vi "Initialize.vi"(8 "error in (no error)":errorcluster, 10 "logger name":string, 11 "file handler in":refnum<class "File Handler.lvclass">) -> (0 "error out":errorcluster, 2 "handler name":string, 3 "file handler out":refnum<class "File Handler.lvclass">)   [LabVIEW 2018, in "GLog.lvlib" / "File Handler.lvclass"]
uses:
  File Handler.lvclass
  File Handler.lvclass/File Handler.ctl
  Send Update Event.vi
  extension/formatting_handler_interface/Formatting Handler.lvclass
  RolloverTrigger/RolloverTrigger.lvclass
  dependencies/Utilities/Utilities.lvlib
panel:
  # "Connector Pane"
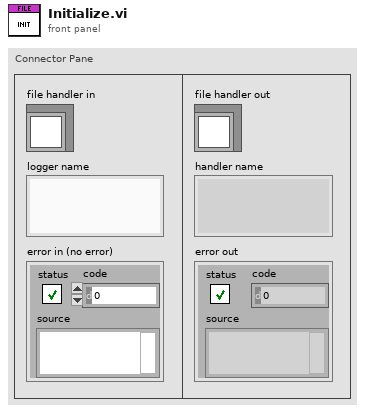
[diagram p1: front panel]
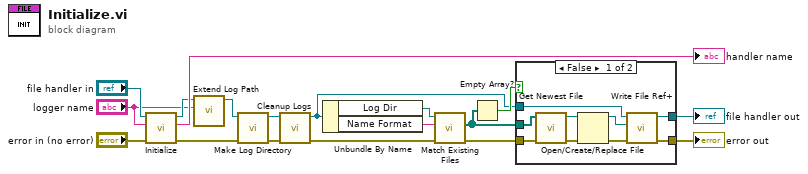
[diagram p0: block diagram]
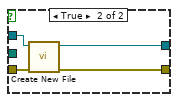
[diagram p2: hidden frame]
diagram:
  n1 = call-parent "Initialize.vi"("error in (no error)"="error in (no error)", "logger name"="logger name", "handler in"="file handler in") -> ("error out"=w3:errorcluster, "handler name"=→"handler name":string, "handler out"=w5:refnum<class "File Handler.lvclass">)  [unwired: 6 in]
  n2 = call "Extend Log Path.vi"("logger name"="logger name", "File Handler in"=w5) -> ("File Handler out"=w2:refnum<class "File Handler.lvclass">)  [unwired: 9 in]
  n3 = call "Make Log Directory.vi"("error in (no error)"=w3, "File Handler in"=w2) -> ("error out"=w18:errorcluster, "dup File Handler"=w1:refnum<class "File Handler.lvclass">)  [unwired: 8 in]
  n4 = call "Cleanup Logs.vi"("error in (no error)"=w18, "file handler in"=w1) -> ("error out"=w12:errorcluster, "file handler out"=w11:refnum<class "File Handler.lvclass">)  [unwired: 8 in]
  n5 = Unbundle By Name(w11) -> ("Log Dir"=w8:path, "Name Format"=w9:string)
  n6 = call "Match Existing Files.vi"("error in (no error)"=w12, "filename format"=w9, "directory in"=w8) -> ("error out"=w10:errorcluster, "matching filenames"=w13:path[])  [unwired: 6 in, 1 out]
  n7 = Empty Array?(array=w13) -> (empty?=w14:bool)
  n8 = case shown="False" w14 {
    tunnel: w13 -> [w27 _]
    tunnel: w11 -> [w24 w29]
    tunnel: [w23 w31] -> w6
    tunnel: [w22 w30] -> w7
    tunnel: w10 -> [w21 w28]
    frame False {
      n9 = call "Get Newest File.vi"("error in (no error)"=w21, "files"=w27) -> ("error out"=w20:errorcluster, "newest file"=w26:path)  [unwired: 8 in]
      n10 = Open/Create/Replace File(file path (use dialog)=w26, error in=w20) -> (refnum out=w25:refnum<file>, error out=w19:errorcluster)  [unwired: 4 in, 1 out]
      n11 = call "Write File Ref+.vi"("error in (no error)"=w19, "File Ref"=w25, "File Handler in"=w24) -> ("error out"=w22:errorcluster, "File Handler out"=w23:refnum<class "File Handler.lvclass">)  [unwired: 7 in]
    }
    frame True {
      n12 = call "Create New File.vi"("error in (no error)"=w28, "file handler in"=w29) -> ("error out"=w30:errorcluster, "file handler out"=w31:refnum<class "File Handler.lvclass">)  [unwired: 8 in]
    }
  }
  "error out" <- w7
  "file handler out" <- w6
